vi "DVR Get Languages.vi"(8 "error in (no error)":errorcluster) -> (0 "error out":errorcluster, 1 "Unicode":string[](array[string]), 2 "ANSI":string[](array[string]), 3 "Languages":string[](array[string]))   [LabVIEW 2019, in "Language Selection.lvlib"]
doc: "Converts the Data Value Reference back into Controls translation.\n- - -\nCopyright (c) 2026, Merecs Engineering GmbH"
uses:
  Language Selection.lvlib
  Global Language Selection.vi
panel:
  # "Connector Pane"
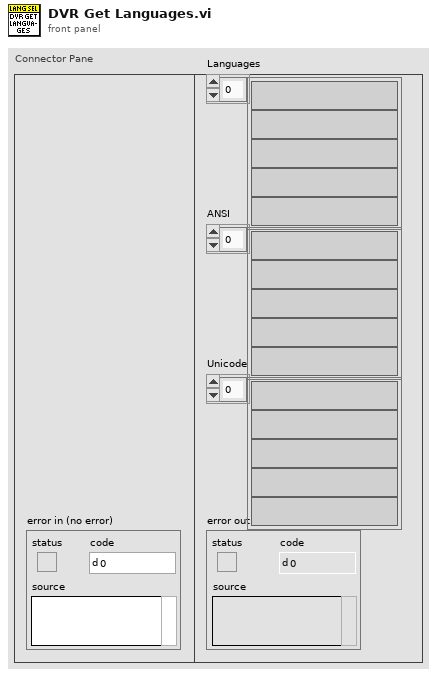
[diagram p1: front panel]
types:
  T1 = typedef "Language Selection.lvlib/Cluster DVR.ctl" = cluster{"Data":T2, "VIs":path[], "FP Translation":map{string, T3}, "Text Translation":map{string, T3}, "Front panels":set{refnum<vi>}}
  T2 = typedef "Language Selection.lvlib/Cluster Settings Data.ctl" = cluster{"Startup Language":string, "Default Language":string, "Languages":cluster{"ANSI":string[], "Unicode":string[]}}
  T3 = typedef "Language Selection.lvlib/Cluster LanguageClusterWithRefnum.ctl" = cluster{"Property":T4[], "Controls":set{refnum<vi>}}
  T4 = typedef "Language Selection.lvlib/Cluster PropertyTranslation.ctl" = cluster{"Type":T5, "Translation ANSI":string[], "Translation Unicode":string[]}
  T5 = typedef "Language Selection.lvlib/Enum Property Type.ctl" = enum16{"NA", "Caption", "String Value", "Boolean Text", "Ring Strings", "1D Array Elements", "2D Array Elements", "(MC)Listbox Header", "(MC)Listbox Items", "Tab Pages Names", "X & Y GraphChart", "Plot Names", "Table Headers", "Table Items", "TipStrip", "Combobox Strings", "Cursor Name", "Tree Col Headers"}
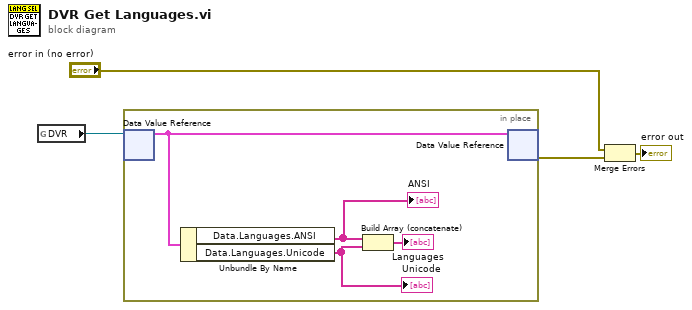
[diagram p0: block diagram]
diagram:
  n1 = global read "Global Language Selection.vi" "DVR"() -> (w1:refnum<data-value>)
  n2 = in-place "In Place Element Structure" {
    n3 = in-place-dvr #1(w1) -> (w8:T1)  [unwired: 1 out]
    n4 = Unbundle By Name(w8) -> ("Data.Languages.ANSI"=w7:string[], "Data.Languages.Unicode"=w6:string[])
    "ANSI" <- w7
    "Unicode" <- w6
    n5 = Build Array (concatenate)(w7, w6) -> (→"Languages":string[])
    n6 = in-place-dvr #1(w8) -> (w3:errorcluster)  [unwired: 1 out]
  }
  n7 = Merge Errors("error in (no error)", w3) -> (→"error out":errorcluster)
